vi "RDC-Lin-Find_eff_length.vi"(9 "Probe Parameters":T2={"lenght [mm]"=50.0, "Core Diameter [mm]"=0.93, "Inner Diameter [mm]"=3.5, "Dieletrisk constant"=2.53}, 10 "Short Probe reading":T1={"Frequency"=array[2001 elements], "Reflection'"=array[2001 elements], "Reflection''"=array[2001 elements], "Permativity'"=array[2001 elements], "Permativity''"=array[2001 elements], "Conductivity"=array[2001 elements], "Loss Tangent"=array[2001 elements], "Resistance"=[], "Reactance"=[]}) -> (1 "Comp Probe K":dbl, 2 "Lenght":dbl format="%#_6e")   [LabVIEW 2020, in "RDC-Reflection_Data_Computation.lvlib"]
doc: "Finds the effective probe length from a short-probe Common Format cluster and the probe parameters, using RDC-Lin-Find_tau and RDC-Probe-Calculate_Constants. Returns Lenght and the compensated probe constant K."
uses:
  RDC-Reflection_Data_Computation.lvlib
  RDC-Probe_parameters.ctl
  Reflector/RFH-common_data_format.ctl
  Reflector/RFH-Reflection_File_Handler.lvlib
panel:
  out "Probe Constant K":dbl
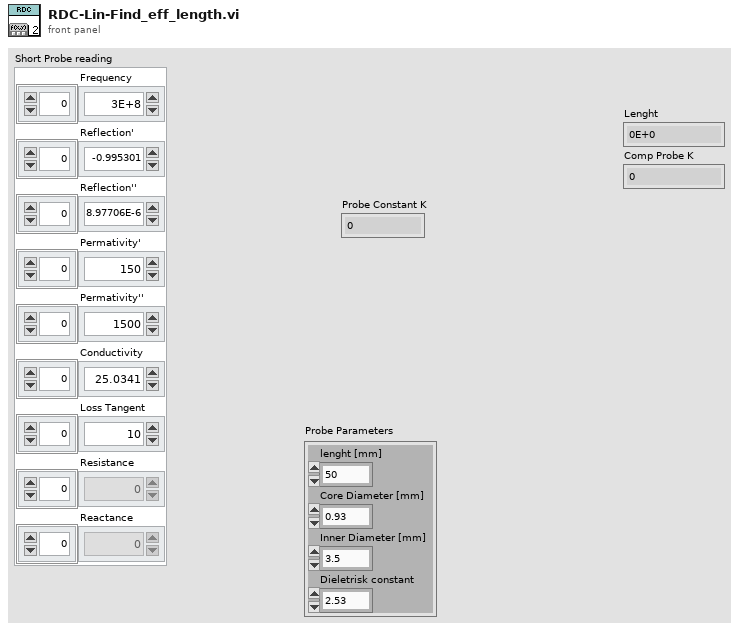
[diagram p1: front panel]
types:
  T1 = typedef "RFH-Reflection_File_Handler.lvlib/RFH-common_data_format.ctl" = cluster{"Frequency":dbl[], "Reflection'":dbl[], "Reflection''":dbl[], "Permativity'":dbl[], "Permativity''":dbl[], "Conductivity":dbl[], "Loss Tangent":dbl[], "Resistance":dbl[], "Reactance":dbl[]}
  T2 = typedef "RDC-Reflection_Data_Computation.lvlib/RDC-Probe_parameters.ctl" = cluster{"lenght [mm]":dbl, "Core Diameter [mm]":dbl, "Inner Diameter [mm]":dbl, "Dieletrisk constant":dbl}
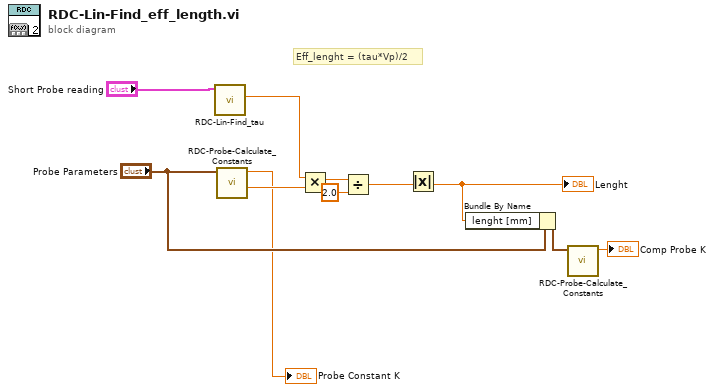
[diagram p0: block diagram]
diagram:
  # "Eff_lenght = (tau*Vp)/2"
  n1 = call "RDC-Lin-Find_tau.vi"("Short Probe reading"="Short Probe reading") -> ("Tau"=w7:dbl)  [unwired: 9 in, 1 out]
  n2 = call "RDC-Probe-Calculate_Constants.vi"("Probe Parameters"="Probe Parameters") -> ("Vp"=w8:dbl, "Probe Constant K"=→"Probe Constant K":dbl)  [unwired: 8 in, 1 out]
  n3 = Multiply(x=w7, y=w8) -> (x*y=w11:dbl)
  n4 = Divide(x=w11, y=2.0) -> (x/y=w9:dbl)
  n5 = Absolute Value(x=w9) -> (abs(x)=w4:dbl)
  "Lenght" <- w4
  n6 = Bundle By Name(cluster="Probe Parameters", "lenght [mm]"=w4) -> (w5:T2)
  n7 = call "RDC-Probe-Calculate_Constants.vi"("Probe Parameters"=w5) -> ("Probe Constant K"=→"Comp Probe K":dbl)  [unwired: 8 in, 2 out]
